vi "Create.vi"(8 "error in (no error)":errorcluster, 11 "CIFPlugin in":refnum<class "CAN_Writer_CANsub_Plugin.lvclass">) -> (0 "error out":errorcluster, 3 "CIFPlugin out":refnum<class "CAN_Writer_CANsub_Plugin.lvclass">)   [LabVIEW 2021, in "CAN_Writer_CANsub_Plugin.lvclass"]
uses:
  CAN_Writer_CANsub_Plugin.lvclass
  CAN_Writer_CANsub_Plugin.lvclass/CAN_Writer_CANsub_Plugin.ctl
  Common/CAN_Writer_CANsub_Common.lvlib
  <vilib>/CIF Foundation/CIF Core/CIFCore/Class/CIFCorePlugin.lvclass
  <vilib>/CIF Foundation/CIF Channels Core/CIFChannels/CIFChannels.lvclass
  <vilib>/CIF Foundation/CIF Core/CIFCore/Common/Typedef/Timing Overrides.ctl
  <vilib>/CIF Foundation/CIF Core/CIFCore/Common/CIFCoreCommon.lvlib
  C:/Program Files/National Instruments/LabVIEW 2021/vi.lib/CIF Foundation/CIF Core/CIFCore/Class/CIFCorePlugin.lvclass
  <vilib>/CIF Foundation/CIF CAN RW Core/typedef/Communication State.ctl
  <vilib>/CIF Foundation/CIF CAN RW Core/CAN_RW_CORE.lvclass
  <vilib>/CIF Foundation/CIF CAN RW Core/typedef/Last Error.ctl
  <vilib>/CIF Foundation/CIF CAN RW Core/typedef/CAN Status.ctl
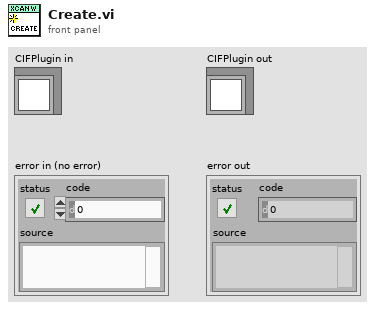
[diagram p1: front panel]
types:
  T1 = typedef "CAN_RW_CORE.lvclass/CAN Status.ctl" = cluster{"Comm State":T2, "Last Error":T3, "RX Error Counter":u8, "TX Error Counter":u8}
  T2 = typedef "CAN_RW_CORE.lvclass/Communication State.ctl" = enum16{"Error Active", "Error Passive", "Bus Off"}
  T3 = typedef "CAN_RW_CORE.lvclass/Last Error.ctl" = enum16{"None", "Stuff", "Form", "Ack", "Bit1", "Bit0", "CRC", "Unknown"}
  T4 = typedef "CIFCoreCommon.lvlib/Timing Overrides.ctl" = cluster{"Override Timing":bool, "Skip Sleep":bool, "Period (s)":dbl}
  T5 = typedef "ChannelRegistrar.lvlib/Channel Definition.ctl" = cluster{"Name":string, "Direction":T6, "Type":T7, "Custom Config Data":u8[]}
  T6 = typedef "ChannelCommon.lvlib/Direction.ctl" = enum8{"Publisher", "Subscriber"}
  T7 = typedef "ChannelRegistrar.lvlib/Registered Channel Types.ctl" = enum8{"Custom", "Double_Tag", "I64_Tag", "U64_Tag", "U8_FIFO", "CAN_FIFO", "L2Enet_FIFO", "DAQ_FIFO", "Universal_FIFO", "String_Tag"}
  T8 = typedef "CIFCorePlugin.lvclass/Running Internal Data.ctl" = cluster{"Refresh":bool, "Iterations":i64, "Housekeep only":bool, "Configured period (ns)":i64, "Update channel OOB":bool, "Configuration Change":bool, "Disable Auto Benchmark":bool, "gRPC Loop":bool, "Timed Loop Supported":bool, "Windows Late Cycle Warning":bool, "Prepared":bool}
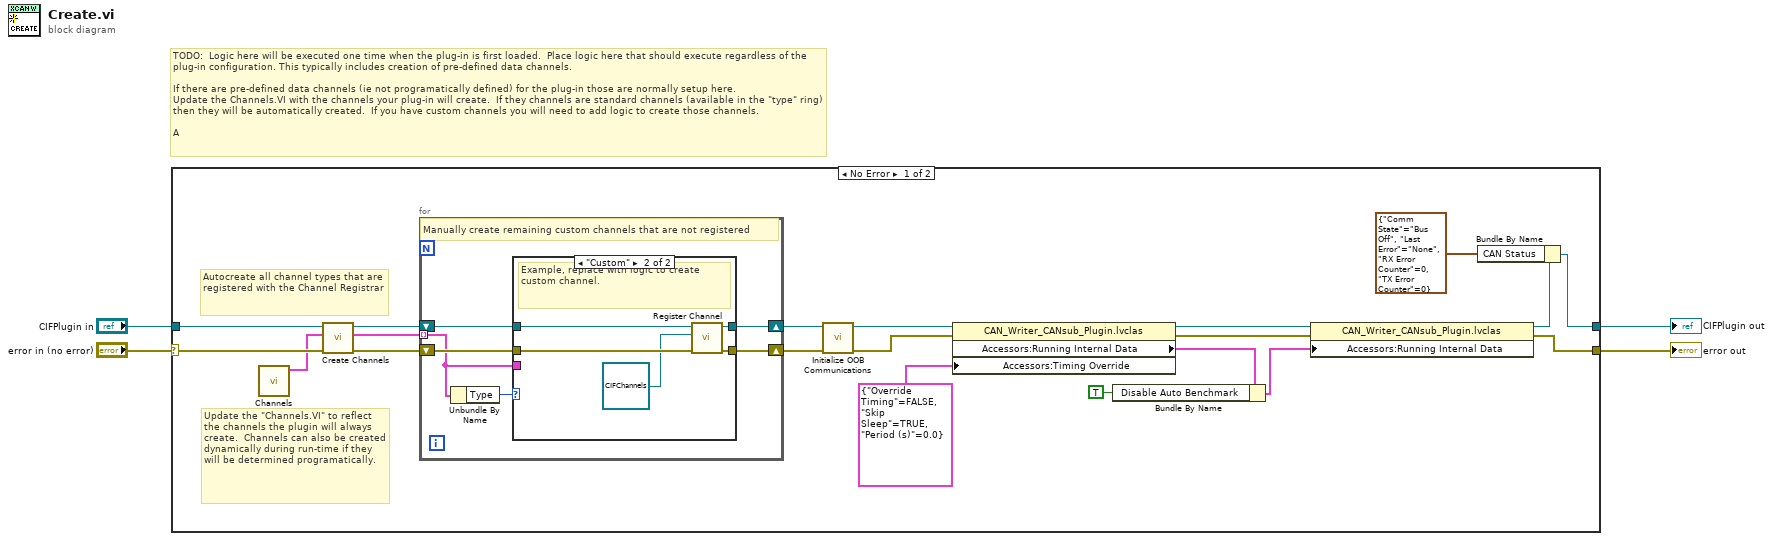
[diagram p0: block diagram]
diagram:
  # "TODO:  Logic here will be executed one time when the plug-in is first loaded.  Place logic here that should execute regardless of the plug-in configuration. This typically includes creation of pre-defined data channels.\n\nIf there are pre-defined data channels (ie not programatically defined) for the plug-in those are normally setup here.  \nUpdate the Channels.VI with the channels your plug-in will create.  If they channels are standard channels (available in the \"type\" ring) then they will be automatically created.  If you have custom channels you will need to add logic to create those channels.\n\nA"
  n1 = case shown="No Error" "error in (no error)" {
    selector: "error in (no error)" -> [w23 w39]
    tunnel: [w11 w39] -> w1
    tunnel: [w6 w38] -> w2
    tunnel: "CIFPlugin in" -> [w24 w38]
    frame No Error {
      # "Update the \"Channels.VI\" to reflect the channels the plugin will always create.  Channels can also be created dynamically during run-time if they will be determined programatically."
      # "Autocreate all channel types that are registered with the Channel Registrar"
      n2 = call "Channels.vi"() -> ("Channels to Create"=w22:T5[])  [unwired: 10 in, 1 out]
      n3 = call <vilib>:"Create Channels.vi"("error in (no error)"=w23, "Channels to Create in"=w22, "CIFCorePlugin in"=w24) -> ("error out"=w19:errorcluster, "Channels to Create out"=w21:T5[], "CIFCorePlugin in"=w20:refnum<class "CAN_Writer_CANsub_Plugin.lvclass">)  [unwired: 6 in]
      n4 = for {
        tunnel: w21 -> [w25] mode=indexing
        shift-right: [w28] -> w18
        shift-left: w20 -> [w30]
        shift-right: [w27] -> w17
        shift-left: w19 -> [w29]
        # "Manually create remaining custom channels that are not registered"
        n5 = Unbundle By Name(w25) -> ("Type"=w26:T7)
        n6 = case shown="\"Custom\"" w26 {
          tunnel: w30 -> [w32 w37]
          tunnel: w29 -> [w31 w36]
          tunnel: [w32 w35] -> w28
          tunnel: [w31 w34] -> w27
          tunnel: w25 -> [_ _]
          frame Default {
          }
          frame "Custom" {
            # "Example, replace with logic to create custom channel."
            n7 = call <vilib>:"Register Channel.vi"("error in (no error)"=w36, "Channel"=refnum<class "CIFChannels.lvclass"> refnum, "CIFCorePlugin in"=w37) -> ("error out"=w34:errorcluster, "CIFCorePlugin in"=w35:refnum<class "CAN_Writer_CANsub_Plugin.lvclass">)  [unwired: 7 in]
          }
        }
      }
      n8 = call "Initialize OOB Communications.vi"("error in (no error)"=w17, "CIFPlugin in"=w18) -> ("error out"=w15:errorcluster, "CIFPlugin out"=w16:refnum<class "CAN_Writer_CANsub_Plugin.lvclass">)  [unwired: 8 in]
      n9 = property class="CAN_Writer_CANsub_Plugin.lvclas"(reference=w16, error in=w15, "Accessors:Timing Override"=T4 {"Override Timing"=FALSE, "Skip Sleep"=TRUE, "Period (s)"=0.0} ("Timing Override")) -> (reference out=w13:refnum<class "CAN_Writer_CANsub_Plugin.lvclass">, error out=w12:errorcluster, "Accessors:Running Internal Data"=w10:T8)
      n10 = Bundle By Name(cluster=w10, "Disable Auto Benchmark"=TRUE) -> (w8:T8)
      n11 = property class="CAN_Writer_CANsub_Plugin.lvclas"(reference=w13, error in=w12, "Accessors:Running Internal Data"=w8) -> (reference out=w7:refnum<class "CAN_Writer_CANsub_Plugin.lvclass">, error out=w11:errorcluster)
      n12 = Bundle By Name(cluster=w7, "CAN Status"=T1 {"Comm State"=enum."Bus Off", "Last Error"=enum."None", "RX Error Counter"=0, "TX Error Counter"=0} ("-> gRPC Comm.Cyclic Data -> gRPC .CAN Status")) -> (w6:refnum<class "CAN_Writer_CANsub_Plugin.lvclass">)
    }
    frame Error {
    }
  }
  "CIFPlugin out" <- w2
  "error out" <- w1
